vi "AdaptToInputs.vi"(3 "Term Types":T1[](array[typedef]), 4 "XRef":refnum<vi>, 5 "State In":T4) -> (0 "Reply":string[](array[string]), 2 "State Out":T4)   [LabVIEW 2012, in "Minimum Array Size.xnode"]
uses:
  Minimum Array Size.xnode
  State.ctl
  <vilib>/XNodeSupport/XNodeTermTypeIDPair.ctl
  <vilib>/XNodeSupport/XNodeType.ctl
  <vilib>/XNodeSupport/XNodeString.ctl
  <userlib>/_LAVAcr/Scripting Tools/XNode Support/Find term type by ID_type.vi
  <vilib>/Utility/VariantDataType/VariantType.lvlib
  <userlib>/_LAVAcr/Scripting Tools/XNode Support/XNode Support.lvlib
  <vilib>/XNodeSupport/NI_XNodeSupport.lvlib
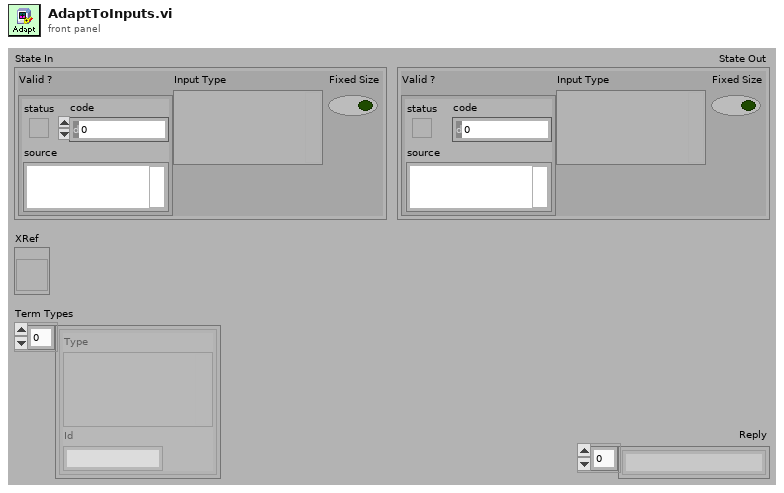
[diagram p1: front panel]
types:
  T1 = typedef "NI_XNodeSupport.lvlib/XNodeTermTypeIDPair.ctl" = cluster{"Type":T2, "Id":T3}
  T2 = typedef "NI_XNodeSupport.lvlib/XNodeType.ctl" = variant
  T3 = typedef "NI_XNodeSupport.lvlib/XNodeString.ctl" = string
  T4 = typedef "Minimum Array Size.xnode/State.ctl" = cluster{"Valid ?":errorcluster, "Input Type":variant, "Fixed Size":bool}
  T5 = typedef "VariantType.lvlib/Type.ctl" = enum8{"Invalid Type", "Void", "I8", "I16", "I32", "I64", "U8", "U16", "U32", "U64", "Single Float", "Double Float", "Extended Float", "Single Complex", "Double Complex", "Extended Complex", "Enum U8", "Enum U16", "Enum U32", "Enum U64", "Single Float With Unit", "Double Float With Unit", "Extended Float With Unit", "Single Complex with Unit", "Double Complex with Unit", "Extended Complex with Unit", "Boolean", "String", "Path", "Picture", "Tag", "Array", "Cluster", "Variant", "LV Variant", "Waveform", "Timestamp", "Digital Waveform", "Digital Data", "ExpressData", "Refnum", "External Data", "VI", "Poly VI", "LabVIEW Class Instance", "Fixed Point"}
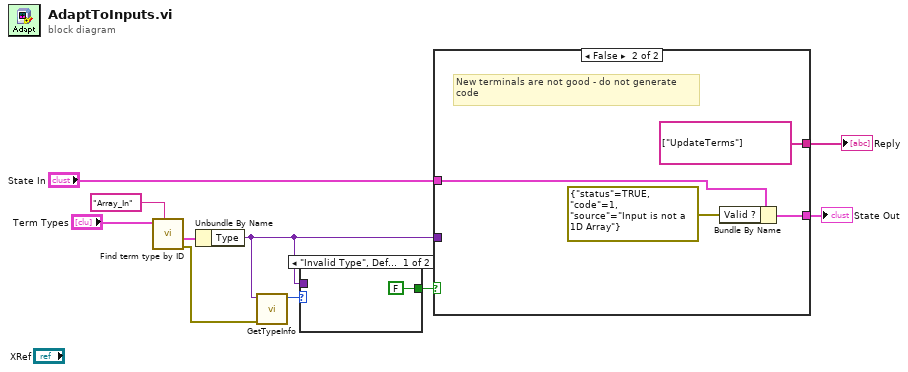
[diagram p0: block diagram]
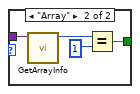
[diagram p2: hidden frame]
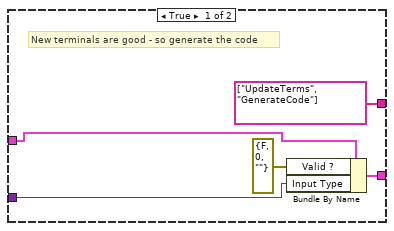
[diagram p3: hidden frame]
diagram:
  n1 = call-poly <userlib>:"Find term type by ID.vi"("Search ID"="Array_In", "Term Types"="Term Types") -> ("error out"=w5:errorcluster, "Term Type"=w4:T1)  [unwired: 1 in, 7 out]
  n2 = Unbundle By Name(w4) -> ("Type"=w2:T2)
  n3 = call <vilib>:"GetTypeInfo.vi"("error in (no error)"=w5, "Variant"=w2) -> ("Type Enum"=w3:T5)  [unwired: 9 out]
  n4 = case shown="\"Invalid Type\", Default" w3 {
    tunnel: w2 -> [_ w15]
    tunnel: [FALSE w12] -> w1
    frame "Invalid Type", Default {
    }
    frame "Array" {
      n5 = call <vilib>:"GetArrayInfo.vi"("Variant"=w15) -> ("NDims"=w14:i32)  [unwired: 1 in, 9 out]
      n6 = Equal?(x=w14, y=1) -> (x = y?=w12:bool)
    }
  }
  n7 = case shown="False" w1 {
    tunnel: "State In" -> [w20 w24]
    tunnel: [w18 w22] -> w9
    tunnel: [string[] ["UpdateTerms", "GenerateCode"] ("Reply") string[] ["UpdateTerms"] ("Reply")] -> w8
    tunnel: w2 -> [w16 _]
    frame True {
      # "New terminals are good - so generate the code"
      n8 = Bundle By Name(cluster=w20, "Valid ?"=errorcluster {"status"=FALSE, "code"=0, "source"=""}, "Input Type"=w16) -> (w18:T4)
    }
    frame False {
      # "New terminals are not good - do not generate\ncode"
      n9 = Bundle By Name(cluster=w24, "Valid ?"=errorcluster {"status"=TRUE, "code"=1, "source"="Input is not a 1D Array"}) -> (w22:T4)
    }
  }
  "Reply" <- w8
  "State Out" <- w9
